vi "GpuMat CopyTo.vi"(6 "Mask in":refnum<class "GpuMat.lvclass">, 8 "error in (no error)":errorcluster, 9 "Stream in":refnum<class "Stream.lvclass">, 10 "Dst in":refnum<class "GpuMat.lvclass">, 11 "Src in":refnum<class "GpuMat.lvclass">) -> (0 "error out":errorcluster, 1 "Stream out":refnum<class "Stream.lvclass">, 3 "Dst out":refnum<class "GpuMat.lvclass">)   [LabVIEW 2020, in "OpenLvVision_OpenCv.lvlib" / "Cuda.lvlib" / "GpuMat.lvclass"]
doc: "Copies the matrix data from a source GpuMat to a destination GpuMat. \nIf the destination matrix does not have the matching size and data type, it is automatically reallocated before the copy occurs."
uses:
  GpuMat.lvclass
  OpenLvVision_OpenCv.lvlib
  <vilib>/Utility/error.llb/Error Cluster From Error Code.vi
  <vilib>/ErrorRing/Error Ring.xnode
  _LvHelpers/EdvrObject/EdvrObject.lvclass
  Dlls/OlvOpenCvWrapper.dll
  C:/Users/lukas/Documents/OpenLvVision_OpenCv/SourceCode/LabView/OpenLvVision_OpenCv/_LvHelpers/EdvrObject/EdvrObject.lvclass
  Stream/Stream.lvclass
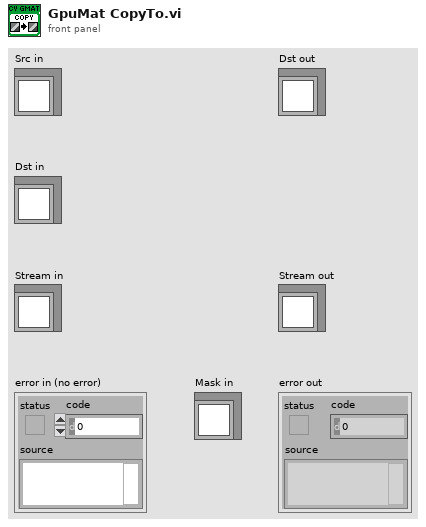
[diagram p1: front panel]
types:
  T1 = typedef "OpenLvVision_OpenCv.lvlib/EdvrObject.lvclass/Edvr.ctl" = refnum<data-value>
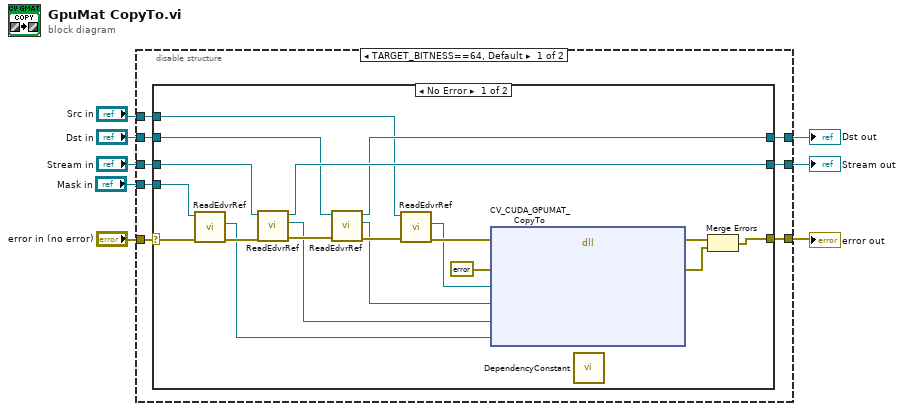
[diagram p0: block diagram]
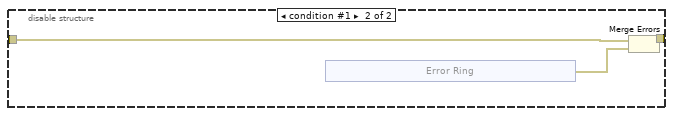
[diagram p3: hidden frame]
diagram:
  n1 = disable-structure shown="TARGET_BITNESS==64, Default" {
    disable-tunnel: "error in (no error)" -> [w16 w40]
    disable-tunnel: [w15 w41] -> w8
    disable-tunnel: "Src in" -> [w14 _]
    disable-tunnel: [w13 _] -> w2
    disable-tunnel: "Stream in" -> [w12 _]
    disable-tunnel: [w11 _] -> w4
    disable-tunnel: "Dst in" -> [w10 _]
    disable-tunnel: "Mask in" -> [w9 _]
    frame condition #0 (active) {
      n2 = case shown="No Error" w16 {
        selector: w16 -> [w20 w38]
        tunnel: [w30 w38] -> w15
        tunnel: w14 -> [w21 _]
        tunnel: [w22 w36] -> w13
        tunnel: w12 -> [w24 w37]
        tunnel: [w25 w37] -> w11
        tunnel: w10 -> [w23 w36]
        tunnel: w9 -> [w18 _]
        frame No Error {
          n3 = call "ReadEdvrRef.vi"("error in (no error)"=w20, "EdvrObject in"=w18) -> ("error out"=w19:errorcluster, "Edvr"=w17:T1)  [unwired: 7 in, 1 out]
          n4 = call "ReadEdvrRef.vi"("error in (no error)"=w19, "EdvrObject in"=w24) -> ("error out"=w27:errorcluster, "Edvr"=w26:T1, "EdvrObject out"=w25:refnum<class "Stream.lvclass">)  [unwired: 7 in]
          n5 = call "ReadEdvrRef.vi"("error in (no error)"=w27, "EdvrObject in"=w23) -> ("error out"=w29:errorcluster, "Edvr"=w28:T1, "EdvrObject out"=w22:refnum<class "GpuMat.lvclass">)  [unwired: 7 in]
          n6 = call "ReadEdvrRef.vi"("error in (no error)"=w29, "EdvrObject in"=w21) -> ("error out"=w32:errorcluster, "Edvr"=w31:T1)  [unwired: 7 in, 1 out]
          n7 = dll-call lib="C:/Users/lukas/Documents/OpenLvVision_OpenCv/SourceCode/LabView/OpenLvVision_OpenCv/Dlls/OlvOpenCvWrapper.dll" fn="CV_CUDA_GPUMAT_CopyTo"(error in=w32, "Error"=errorcluster {"status"=FALSE, "code"=0, "source"=""} ("error out"), "srcRef"=w31, "dstRef"=w28, "streamRef"=w26, "maskRef"=w17) -> (error out=w35:errorcluster, "Error"=w34:errorcluster)  [unwired: 7 in, 1 out]
          n8 = call "DependencyConstant.vi"() -> ()  [unwired: 12 in]
          n9 = Merge Errors(w35, w34) -> (w30:errorcluster)
        }
        frame Error {
        }
      }
    }
    frame condition #1 {
      n10 = xnode "Error Ring"() -> ("error out"=w39:errorcluster)
      n11 = Merge Errors(w40, w39) -> (w41:errorcluster)
    }
  }
  "error out" <- w8
  "Stream out" <- w4
  "Dst out" <- w2
